vi "LHF.DB.Mongo.Util.VariantToFields.vi"(0 "projection type":variant, 5 "error in (no error)":errorcluster) -> (14 "BsonDocument":refnum<k24>, 19 "error out":errorcluster)   [LabVIEW 2013, in "LHF.DB.Mongo.lvclass"]
uses:
  LHF.DB.Mongo.lvclass
  C:/Users/Ricardo/Desktop/Projetos/LabVIEW-MongoDB/src/Driver/MongoDB.Bson.dll
  Driver/MongoDB.Bson.dll
  C:/Users/Ricardo/Desktop/Projetos/LabVIEW-MongoDB/src/Driver/MongoDB.Driver.dll
  Driver/MongoDB.Driver.dll
  <vilib>/Utility/VariantDataType/VariantType.lvlib
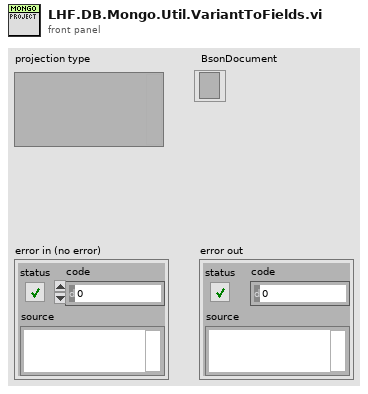
[diagram p1: front panel]
types:
  T1 = typedef "VariantType.lvlib/Type.ctl" = enum8{"Invalid Type", "Void", "I8", "I16", "I32", "I64", "U8", "U16", "U32", "U64", "Single Float", "Double Float", "Extended Float", "Single Complex", "Double Complex", "Extended Complex", "Enum U8", "Enum U16", "Enum U32", "Enum U64", "Single Float With Unit", "Double Float With Unit", "Extended Float With Unit", "Single Complex with Unit", "Double Complex with Unit", "Extended Complex with Unit", "Boolean", "String", "Path", "Picture", "Tag", "Array", "Cluster", "Variant", "LV Variant", "Waveform", "Timestamp", "Digital Waveform", "Digital Data", "ExpressData", "Refnum", "External Data", "VI", "Poly VI", "LabVIEW Class Instance", "Fixed Point"}
  T2 = typedef "LHF.DB.Mongo.lvclass/LHF.DB.Mongo.Typedef.VariantData.ctl" = cluster{"Type Enum":T1, "Name":string, "Variant":variant}
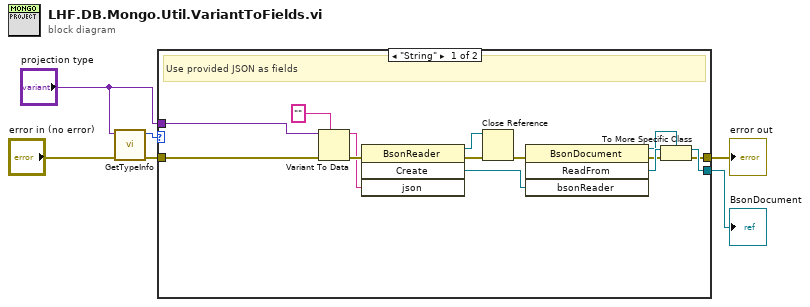
[diagram p0: block diagram]
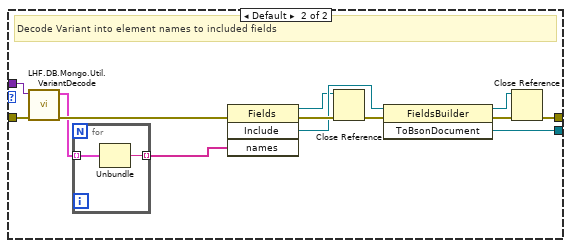
[diagram p2: hidden frame]
diagram:
  n1 = call <vilib>:"GetTypeInfo.vi"("error in (no error)"="error in (no error)", "Variant"="projection type") -> ("error out"=w2:errorcluster, "Type Enum"=w4:T1)  [unwired: 5 in, 3 out]
  n2 = case shown="\"String\"" w4 {
    tunnel: w2 -> [w14 w32]
    tunnel: [w7 w21] -> w1
    tunnel: [w10 w25] -> w6
    tunnel: "projection type" -> [w20 w24]
    frame "String" {
      # "Use provided JSON as fields"
      n3 = Variant To Data(error in=w14, type="", Variant=w20) -> (data=w15:string, error out=w16:errorcluster)
      n4 = invoke class="BsonReader" method="Create"(error in=w16, "json"=w15) -> (reference out=w18:refnum<k24>, error out=w13:errorcluster, "Create"=w17:refnum<k24>)  [unwired: 2 in, 1 out]
      n5 = Close Reference(reference=w18, error in (no error)=w13) -> (error out=w12:errorcluster)
      n6 = invoke class="BsonDocument" method="ReadFrom"(error in=w12, "bsonReader"=w17) -> (reference out=w8:refnum<k24>, error out=w9:errorcluster, "ReadFrom"=w11:refnum<k24>)  [unwired: 2 in, 1 out]
      n7 = To More Specific Class(target class=w8, reference=w11, error in=w9) -> (specific class reference=w10:refnum<k24>, error out=w7:errorcluster)
    }
    frame Default {
      # "Decode Variant into element names to included fields"
      n8 = call "LHF.DB.Mongo.Util.VariantDecode.vi"("error in (no error)"=w32, "variant"=w24) -> ("error out"=w33:errorcluster, "Variant Data"=w30:T2[])  [unwired: 7 in, 1 out]
      n9 = for {
        tunnel: w30 -> [w35] mode=indexing
        tunnel: [w34] -> w31 mode=indexing
        n10 = Unbundle(w35) -> ("Name"=w34:string)  [unwired: 2 out]
      }
      n11 = invoke class="Fields" method="Include"(error in=w33, "names"=w31) -> (reference out=w26:refnum<k24>, error out=w29:errorcluster, "Include"=w28:refnum<k24>)  [unwired: 2 in, 1 out]
      n12 = Close Reference(reference=w26, error in (no error)=w29) -> (error out=w27:errorcluster)
      n13 = invoke class="FieldsBuilder" method="ToBsonDocument"(reference=w28, error in=w27) -> (reference out=w23:refnum<k24>, error out=w22:errorcluster, "ToBsonDocument"=w25:refnum<k24>)  [unwired: 1 in]
      n14 = Close Reference(reference=w23, error in (no error)=w22) -> (error out=w21:errorcluster)
    }
  }
  "error out" <- w1
  "BsonDocument" <- w6
